vi "SMU Level Settings Extract.vi"(0 ".digilevel File Path":path, 9 "Pin Name":string) -> (3 "IRange":dbl, 4 "Vf":dbl, 6 "Ic":dbl, 8 "If":dbl, 10 "Vc":dbl, 14 "VRange":dbl, 15 "Sense":dbl)   [LabVIEW 2025, in "Digital Pattern Sequencer.lvclass"]
uses:
  Digital Pattern Sequencer.lvclass
  Digital Pattern Sequencer.lvclass/Digital Pattern Sequencer.ctl
  <resource>/objmgr/DOMUserDefRef.rc
  <vilib>/xml/NI_XML.lvlib
  <vilib>/xml/Load XML String.vi
  <vilib>/xml/XPath/Get All Matched Nodes (String).vi
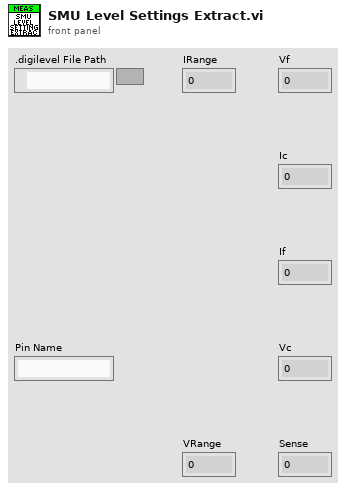
[diagram p1: front panel]
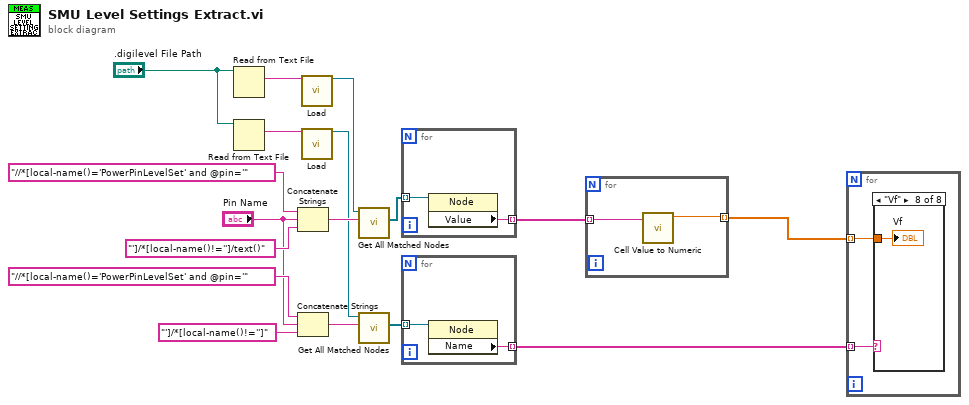
[diagram p0: block diagram]
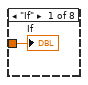
[diagram p2: hidden frame]
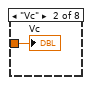
[diagram p3: hidden frame]
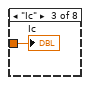
[diagram p4: hidden frame]
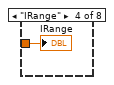
[diagram p5: hidden frame]
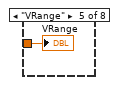
[diagram p6: hidden frame]
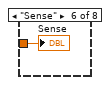
[diagram p7: hidden frame]
diagram:
  n1 = Read from Text File(file (use dialog)=".digilevel File Path") -> (text=w15:string)  [unwired: 3 in, 3 out]
  n2 = Read from Text File(file (use dialog)=".digilevel File Path") -> (text=w8:string)  [unwired: 3 in, 3 out]
  n3 = Concatenate Strings("//*[local-name()='PowerPinLevelSet' and @pin='" ("string"), "Pin Name", "']/*[local-name()!='']/text()" ("string")) -> (w14:string)
  n4 = Concatenate Strings("//*[local-name()='PowerPinLevelSet' and @pin='" ("string"), "Pin Name", "']/*[local-name()!='']" ("string")) -> (w7:string)
  n5 = call-poly <vilib>:"Load.vi"("XML string"=w15) -> ("DOM document out"=w16:refnum<k20>)  [unwired: 12 in, 2 out]
  n6 = call-poly <vilib>:"Load.vi"("XML string"=w8) -> ("DOM document out"=w9:refnum<k20>)  [unwired: 12 in, 2 out]
  n7 = call-poly <vilib>:"Get All Matched Nodes.vi"("XPath expression"=w14, "node in"=w16) -> ("node result array"=w17:refnum<k20>[])  [unwired: 7 in, 2 out]
  n8 = call-poly <vilib>:"Get All Matched Nodes.vi"("XPath expression"=w7, "node in"=w9) -> ("node result array"=w10:refnum<k20>[])  [unwired: 7 in, 2 out]
  n9 = for {
    tunnel: w17 -> [w19] mode=indexing
    tunnel: [w18] -> w11 mode=indexing
    n10 = property class="Node"(reference=w19) -> ("Value"=w18:string)  [unwired: 1 in, 2 out]
  }
  n11 = for {
    tunnel: w10 -> [w21] mode=indexing
    tunnel: [w20] -> w2 mode=indexing
    n12 = property class="Node"(reference=w21) -> ("Name"=w20:string)  [unwired: 1 in, 2 out]
  }
  n13 = for {
    tunnel: w11 -> [w23] mode=indexing
    tunnel: [w22] -> w1 mode=indexing
    n14 = call "Cell Value to Numeric.vi"("Cell Value"=w23) -> ("Numeric"=w22:dbl)  [unwired: 9 in, 1 out]
  }
  n15 = for {
    tunnel: w2 -> [w25] mode=indexing
    tunnel: w1 -> [w24] mode=indexing
    n16 = case shown="\"Vf\"" w25 {
      tunnel: w24 -> [w26 w27 w28 w29 w30 w31 _ w32]
      frame "If" {
        "If" <- w26
      }
      frame "Vc" {
        "Vc" <- w27
      }
      frame "Ic" {
        "Ic" <- w28
      }
      frame "IRange" {
        "IRange" <- w29
      }
      frame "VRange" {
        "VRange" <- w30
      }
      frame "Sense" {
        "Sense" <- w31
      }
      frame Default {
      }
      frame "Vf" {
        "Vf" <- w32
      }
    }
  }
